vi "work1_GetOrder and Cook.vi"() -> ()   [LabVIEW 2020]
panel:
  out "Client Counter":i32
  out "Order ID":i32
  in  "stop":bool
  in  "ID":i32
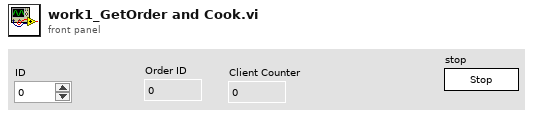
[diagram p1: front panel]
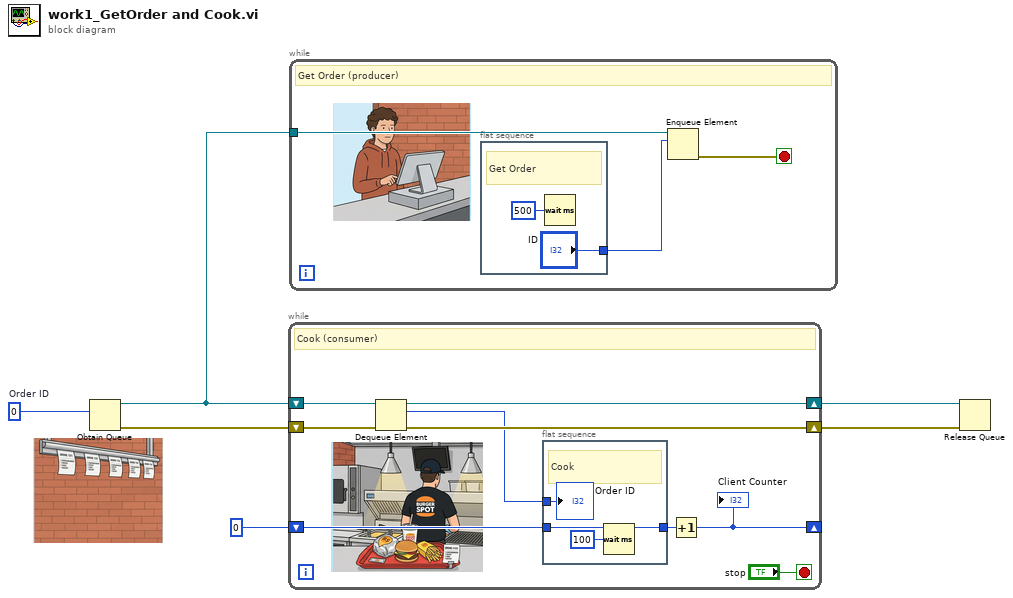
[diagram p0: block diagram]
diagram:
  w2 = 0  # Order ID
  n1 = Obtain Queue(element data type=w2) -> (queue out=w3:refnum<queue>, error out=w6:errorcluster)  [unwired: 4 in, 1 out]
  n2 = while {
    shift-right: [w13] -> w4
    shift-left: w6 -> [w15]
    shift-right: [w14] -> w5
    shift-left: w3 -> [w12]
    shift-right: [w7] -> _
    shift-left: 0 -> [w8]
    stop <- "stop" stop-if-true
    # "Cook (consumer)"
    n3 = Dequeue Element(queue=w12, error in (no error)=w15) -> (queue out=w14:refnum<queue>, element=w11:i32, error out=w13:errorcluster)  [unwired: 1 in, 1 out]
    n4 = flat-sequence {
      tunnel: w11 -> [w17]
      tunnel: [w16] -> w9
      tunnel: w8 -> [w16]
      frame #0 {
        # "Cook"
        n5 = Wait (ms)(milliseconds to wait=u32 100) -> ()  [unwired: 1 out]
        "Order ID" <- w17
      }
    }
    n6 = Increment(x=w9) -> (x+1=w7:i32)
    "Client Counter" <- w7
  }
  n7 = while {
    tunnel: w3 -> [w21]
    stop <- w19 stop-if-true
    # "Get Order (producer)"
    n8 = flat-sequence {
      tunnel: ["ID"] -> w20
      frame #0 {
        # "Get Order"
        n9 = Wait (ms)(milliseconds to wait=u32 500) -> ()  [unwired: 1 out]
      }
    }
    n10 = Enqueue Element(queue=w21, element=w20) -> (error out=w19:errorcluster)  [unwired: 2 in, 2 out]
  }
  n11 = Release Queue(queue=w5, error in (no error)=w4) -> ()  [unwired: 1 in, 3 out]
